vi "GDSProject_GetAllClasses.vi"(1 "AnyProjectItemRefnum":refnum<vi>, 2 "TreeControlRef":refnum<vi>, 3 "ClassProviderName":string, 4 "RootParentTag":string="LabVIEW Object", 5 "error In":errorcluster, 6 "Interfaces(False)":bool, 8 "ClassFilter":string) -> (15 "ClassPaths":path[](array[path]), 16 "ClassTags":string[](array[string]), 19 "error out":errorcluster)   [LabVIEW 2020]
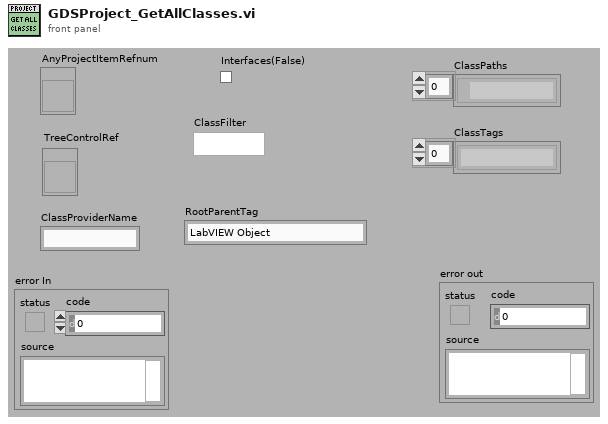
[diagram p1: front panel]
types:
  T1 = cluster{"Classes":refnum<vi>[], "Parents":refnum<vi>[], "ClassIneritance":cluster{string[]}[], "ClassTags":string[], "ClassPaths":path[], "ClassNames":string[]}
  T2 = typedef "GDSLvCLass_ClassSettingsType.ctl" = cluster{"ClassProviderName":string, "ClassTemplateUsed":string, "ClassTemplateVersion":string, "ClassDescription":string, "PlugIns":T3[], "ConnectorPanePattern":string}
  T3 = typedef "GDSLvClass_PlugIn.ctl" = cluster{"Type":T4, "ID":string, "Version":string, "Path":path, "Name":string, "Data":variant}
  T4 = typedef "GDSLvClass_PlugInTypes.ctl" = enum16{"DesignPattern", "MethodTypes"}
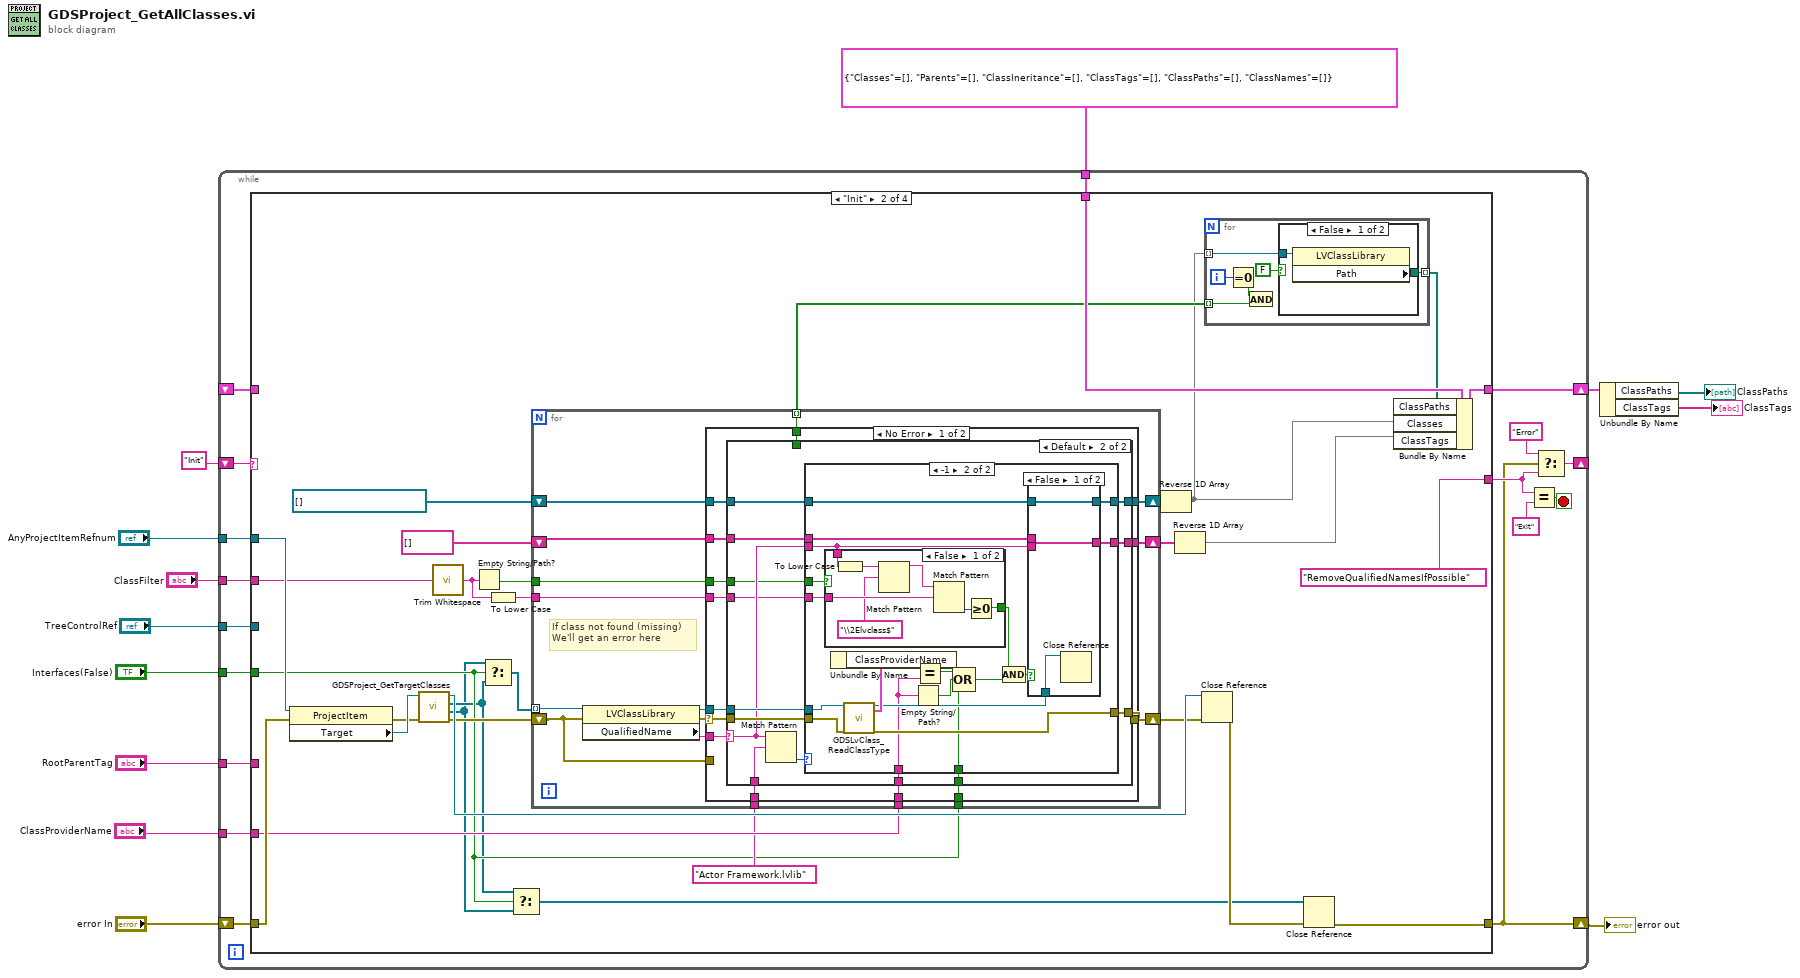
[diagram p0: block diagram]
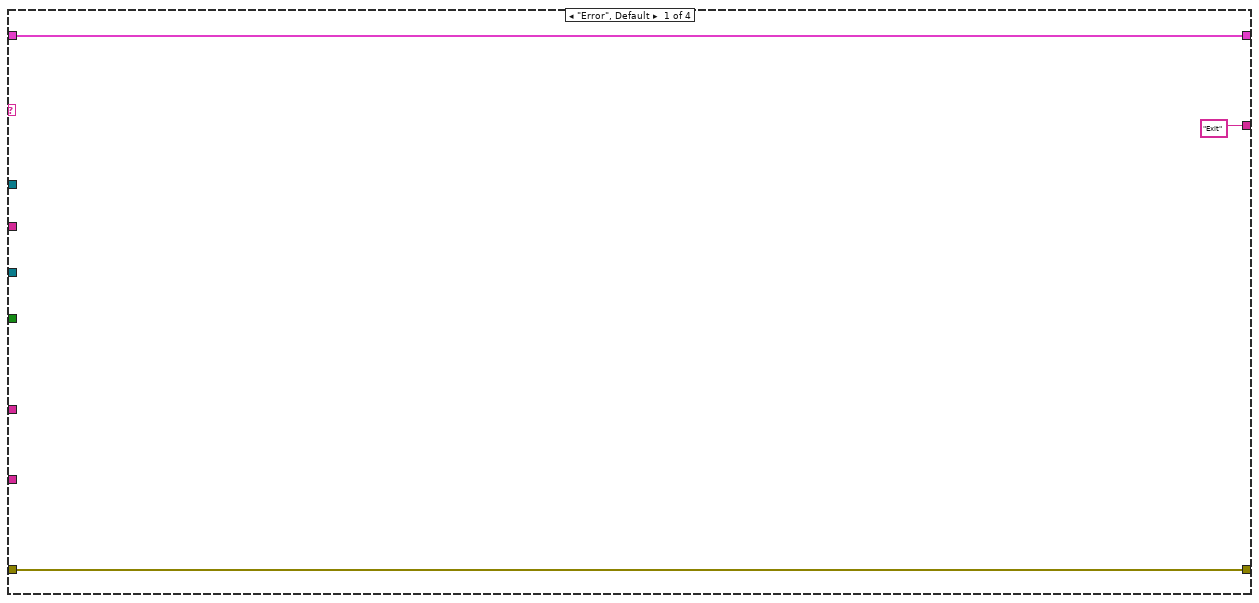
[diagram p2: hidden frame]
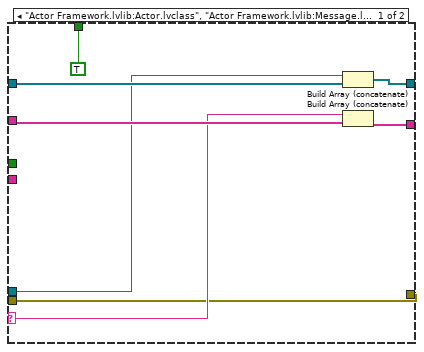
[diagram p4: hidden frame]
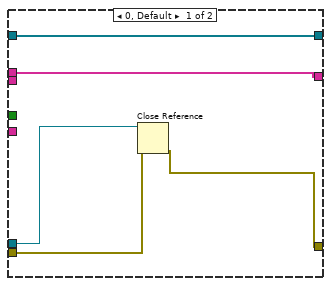
[diagram p5: hidden frame]
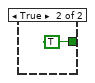
[diagram p6: hidden frame]
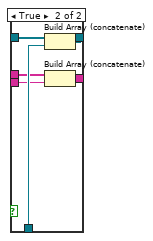
[diagram p7: hidden frame]
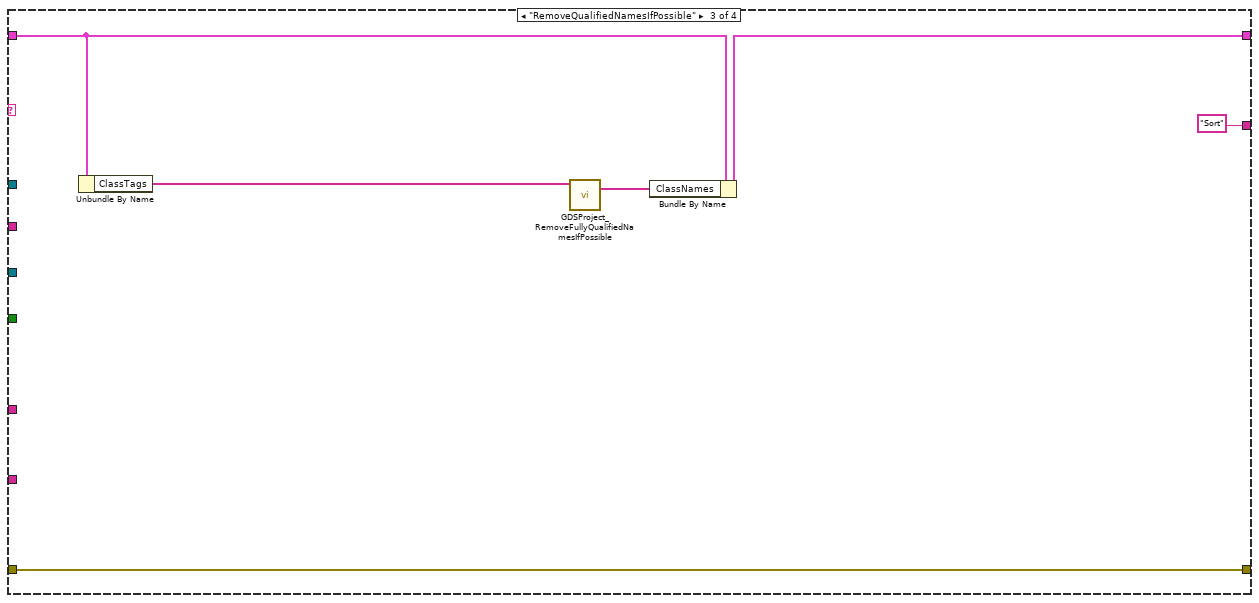
[diagram p9: hidden frame]
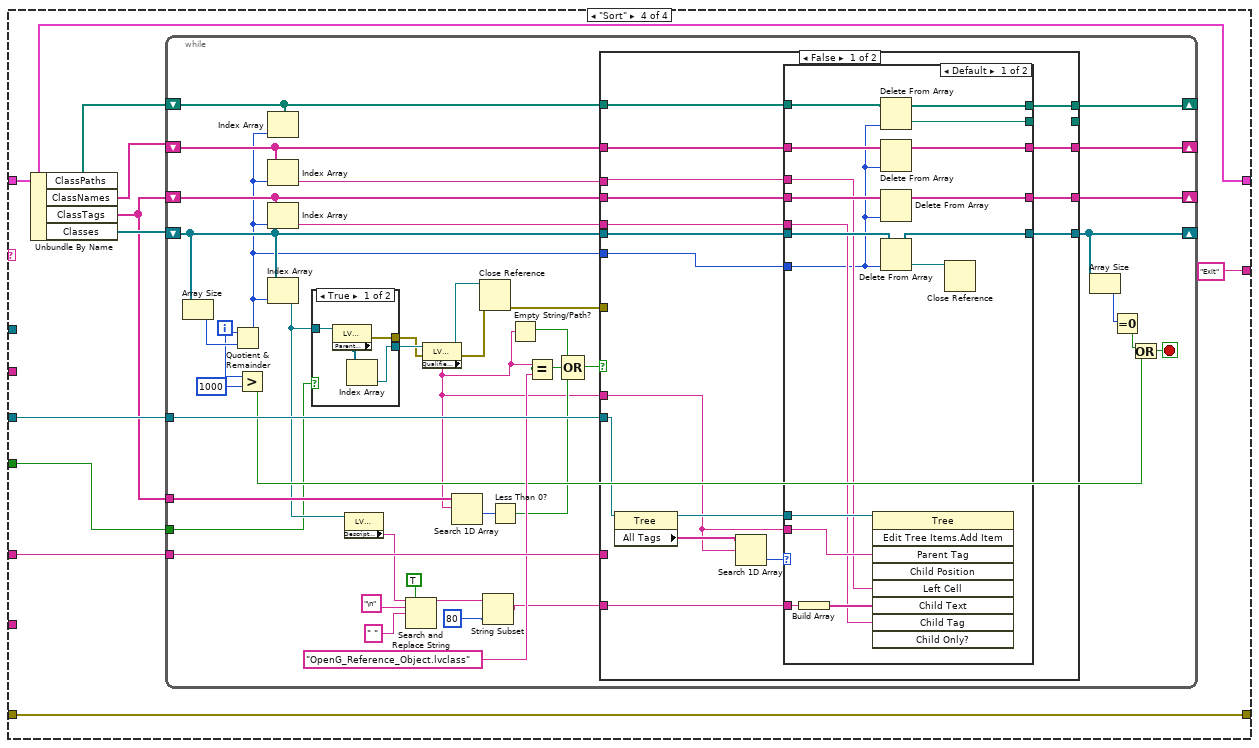
[diagram p10: hidden frame]
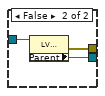
[diagram p11: hidden frame]
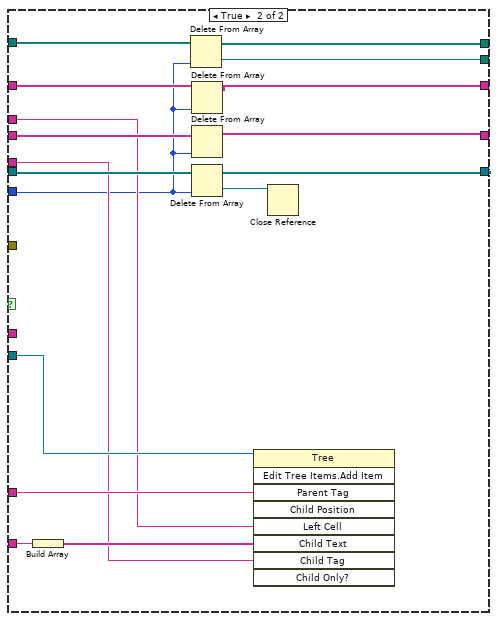
[diagram p13: hidden frame]
diagram:
  n1 = while {
    shift-right: [w23] -> w2
    shift-left: "error In" -> [w30]
    shift-right: [w28] -> _
    shift-left: "Init" -> [w29]
    shift-right: [w22] -> w6
    shift-left: _ -> [w21]
    tunnel: "AnyProjectItemRefnum" -> [w20]
    tunnel: T1 {"Classes"=[], "Parents"=[], "ClassIneritance"=[], "ClassTags"=[], "ClassPaths"=[], "ClassNames"=[]} -> [w19]
    tunnel: "ClassProviderName" -> [w18]
    tunnel: "TreeControlRef" -> [w17]
    tunnel: "RootParentTag" -> [w16]
    tunnel: "Interfaces(False)" -> [w15]
    tunnel: "ClassFilter" -> [w14]
    stop <- w27 stop-if-true
    n2 = case shown="\"Init\"" w29 {
      tunnel: w30 -> [w33 w60 w170 w182]
      tunnel: [w33 w39 w170 w182] -> w23
      tunnel: ["Exit" "RemoveQualifiedNamesIfPossible" "Sort" "Exit"] -> w24
      tunnel: [w31 w58 w172 w180] -> w22
      tunnel: w21 -> [w31 _ w174 w180]
      tunnel: w20 -> [_ w62 _ _]
      tunnel: w19 -> [_ w59 _ _]
      tunnel: w18 -> [_ w57 _ _]
      tunnel: w17 -> [_ _ _ w181]
      tunnel: w16 -> [_ _ _ w183]
      tunnel: w15 -> [_ w43 _ w176]
      tunnel: w14 -> [_ w37 _ _]
      frame "Error", Default {
      }
      frame "Init" {
        n3 = property class="ProjectItem"(reference=w62, error in=w60) -> (error out=w50:errorcluster, "Target"=w51:refnum<vi>)  [unwired: 1 out]
        n4 = call "GDSProject_GetTargetClasses.vi"("error in (no error)"=w50, "TargetItem in"=w51) -> ("error out"=w61:errorcluster, "LvInterfaces"=w41:refnum<vi>[], "LvClasses"=w42:refnum<vi>[], "TargetItem out"=w63:refnum<vi>)  [unwired: 4 in, 2 out]
        n5 = call <vilib>:"Trim Whitespace.vi"("string"=w37) -> ("trimmed string"=w35:string)  [unwired: 1 in]
        n6 = Empty String/Path?(string/path=w35) -> (empty?=w36:bool)
        n7 = Select(t=w41, s=w43, f=w42) -> (s? t:f=w44:refnum<vi>[])
        n8 = To Lower Case(string=w35) -> (all lower case string=w34:string)
        n9 = Select(t=w42, s=w43, f=w41) -> (s? t:f=w38:refnum<vi>[])
        n10 = for {
          tunnel: w44 -> [w77] mode=indexing
          shift-right: [w78] -> w53
          shift-left: refnum<vi>[] [] -> [w88]
          shift-right: [w87] -> w49
          shift-left: w61 -> [w75]
          tunnel: w57 -> [w86]
          shift-right: [w85] -> w54
          shift-left: string[] [] -> [w84]
          tunnel: [w80] -> w48 mode=indexing
          tunnel: "Actor Framework.lvlib" ("Type") -> [w79]
          tunnel: w43 -> [w76]
          tunnel: w36 -> [w74]
          tunnel: w34 -> [w73]
          # "If class not found (missing)\nWe'll get an error here"
          n11 = property class="LVClassLibrary"(reference=w77, error in=w75) -> (reference out=w83:refnum<vi>, error out=w82:errorcluster, "QualifiedName"=w81:string)
          n12 = case shown="No Error" w82 {
            selector: w82 -> [w96 _]
            tunnel: w88 -> [w102 w167]
            tunnel: [w101 w169] -> w87
            tunnel: w86 -> [w100 _]
            tunnel: [w99 w168] -> w85
            tunnel: w84 -> [w98 w168]
            tunnel: w83 -> [w97 _]
            tunnel: w81 -> [w95 _]
            tunnel: [w94 _] -> w80
            tunnel: w79 -> [w93 _]
            tunnel: [w92 w167] -> w78
            tunnel: w76 -> [w91 _]
            tunnel: w75 -> [_ w169]
            tunnel: w74 -> [w90 _]
            tunnel: w73 -> [w89 _]
            frame No Error {
              n13 = case shown="Default" w95 {
                selector: w95 -> [w106 w114]
                tunnel: [w110 w115] -> w92
                tunnel: w102 -> [w104 w124]
                tunnel: [w105 w123] -> w101
                tunnel: w100 -> [_ w122]
                tunnel: [w109 w121] -> w99
                tunnel: w98 -> [w108 w120]
                tunnel: w97 -> [w103 w119]
                tunnel: w96 -> [w105 w118]
                tunnel: [TRUE _] -> w94
                tunnel: w93 -> [_ w117]
                tunnel: w91 -> [_ w113]
                tunnel: w90 -> [_ w112]
                tunnel: w89 -> [_ w111]
                frame "Actor Framework.lvlib:Actor.lvclass", "Actor Framework.lvlib:Message.lvclass" {
                  n14 = Build Array (concatenate)(w103, w104) -> (w110:refnum<vi>[])
                  n15 = Build Array (concatenate)(w106, w108) -> (w109:string[])
                }
                frame Default {
                  n16 = Match Pattern(string=w114, regular expression=w117) -> (offset past match=w116:i32)  [unwired: 1 in, 3 out]
                  n17 = case shown="-1" w116 {
                    tunnel: [w129 w149] -> w115
                    tunnel: w124 -> [w129 w148]
                    tunnel: [w125 w145] -> w123
                    tunnel: w122 -> [_ w143]
                    tunnel: [w128 w140] -> w121
                    tunnel: w120 -> [w128 w139]
                    tunnel: w119 -> [w127 w138]
                    tunnel: w118 -> [w126 w137]
                    tunnel: w114 -> [_ w131]
                    tunnel: w113 -> [_ w136]
                    tunnel: w112 -> [_ w133]
                    tunnel: w111 -> [_ w130]
                    frame 0, Default {
                      n18 = Close Reference(reference=w127, error in (no error)=w126) -> (error out=w125:errorcluster)
                    }
                    frame -1 {
                      n19 = case shown="False" w133 {
                        tunnel: [w153 TRUE] -> w132
                        tunnel: w131 -> [w156 _]
                        tunnel: w130 -> [w155 _]
                        frame False {
                          n20 = To Lower Case(string=w156) -> (all lower case string=w151:string)
                          n21 = Match Pattern(string=w151, regular expression="\\2Elvclass$") -> (before substring=w150:string)  [unwired: 1 in, 3 out]
                          n22 = Match Pattern(string=w150, regular expression=w155) -> (offset past match=w154:i32)  [unwired: 1 in, 3 out]
                          n23 = Greater Or Equal To 0?(x=w154) -> (x >= 0?=w153:bool)
                        }
                        frame True {
                        }
                      }
                      n24 = call "GDSLvClass_ReadClassType.vi"("Class Refnum In"=w138, "error in (no error)"=w137) -> ("Class Refnum Out"=w146:refnum<vi>, "ClassSettings"=w147:T2, "error out"=w145:errorcluster)  [unwired: 15 in]
                      n25 = Unbundle By Name(w147) -> ("ClassProviderName"=w144:string)
                      n26 = Empty String/Path?(string/path=w143) -> (empty?=w141:bool)
                      n27 = Equal?(x=w144, y=w143) -> (x = y?=w142:bool)
                      n28 = Compound Arithmetic op=OR(w142, w141, w136) -> (w135:bool)
                      n29 = Compound Arithmetic op=AND(w132, w135) -> (w134:bool)
                      n30 = case shown="False" w134 {
                        tunnel: [w160 w166] -> w149
                        tunnel: w148 -> [w160 w165]
                        tunnel: w146 -> [w159 w164]
                        tunnel: [w158 w163] -> w140
                        tunnel: w139 -> [w158 w162]
                        tunnel: w131 -> [_ w161]
                        frame False {
                          n31 = Close Reference(reference=w159) -> ()  [unwired: 1 in, 1 out]
                        }
                        frame True {
                          n32 = Build Array (concatenate)(w165, w164) -> (w166:refnum<vi>[])
                          n33 = Build Array (concatenate)(w162, w161) -> (w163:string[])
                        }
                      }
                    }
                  }
                }
              }
            }
            frame Error {
            }
          }
        }
        n34 = Reverse 1D Array(array=w53) -> (reversed array=w47:refnum<vi>[])
        n35 = Reverse 1D Array(array=w54) -> (reversed array=w46:string[])
        n36 = Close Reference(reference=w63, error in (no error)=w49) -> (error out=w40:errorcluster)
        n37 = for {
          tunnel: w47 -> [w70] mode=indexing
          tunnel: [w69] -> w52 mode=indexing
          tunnel: w48 -> [w66] mode=indexing
          i -> [w68]
          n38 = Equal To 0?(x=w68) -> (x = 0?=w67:bool)
          n39 = And(x=w67, y=w66) -> ()  [unwired: 1 out]
          n40 = case shown="False" FALSE {
            tunnel: w70 -> [w72 _]
            tunnel: [w71 _] -> w69
            frame False {
              n41 = property class="LVClassLibrary"(reference=w72) -> ("Path"=w71:path)  [unwired: 1 in, 2 out]
            }
            frame True {
            }
          }
        }
        n42 = Close Reference(reference=w38, error in (no error)=w40) -> (error out=w39:errorcluster)
        n43 = Bundle By Name(cluster=w59, "ClassPaths"=w52, "Classes"=w47, "ClassTags"=w46) -> (w58:T1)
      }
      frame "RemoveQualifiedNamesIfPossible" {
        n44 = Unbundle By Name(w174) -> ("ClassTags"=w175:string[])
        n45 = call "GDSProject_RemoveFullyQualifiedNamesIfPossible.vi"("ItemnamesIn"=w175) -> ("ItemnamesOut"=w173:string[])  [unwired: 10 in]
        n46 = Bundle By Name(cluster=w174, "ClassNames"=w173) -> (w172:T1)
      }
      frame "Sort" {
        n47 = Unbundle By Name(w180) -> ("ClassPaths"=w177:path[], "ClassNames"=w179:string[], "ClassTags"=w178:string[], "Classes"=w185:refnum<vi>[])
        n48 = while {
          shift-right: [w225] -> _
          shift-left: w185 -> [w226]
          tunnel: w181 -> [w227]
          tunnel: w183 -> [w222]
          tunnel: w178 -> [w212]
          shift-right: [w203] -> _
          shift-left: w178 -> [w202]
          shift-right: [w199] -> _
          shift-left: w179 -> [w200]
          shift-right: [w187] -> _
          shift-left: w177 -> [w188]
          tunnel: w176 -> [w186]
          i -> [w215]
          stop <- w216 stop-if-true
          n49 = Array Size(array=w226) -> (size(s)=w223:i32)
          n50 = Quotient & Remainder(x=w215, y=w223) -> (x-y*floor(x/y)=w189:i32)  [unwired: 1 out]
          n51 = Greater?(x=w215, y=1000) -> (0:w213:bool)
          n52 = Index Array(array=w188, index=w189) -> ()  [unwired: 1 out]
          n53 = Index Array(array=w200, index=w189) -> (element=w197:string)
          n54 = Index Array(array=w202, index=w189) -> (element=w201:string)
          n55 = Index Array(array=w226, index=w189) -> (element=w196:refnum<vi>)
          n56 = case shown="True" w186 {
            tunnel: [w228 w234] -> w204
            tunnel: w196 -> [w231 w233]
            tunnel: [w230 w232] -> w193
            frame True {
              n57 = property class="LVClassLibrary"(reference=w231) -> (error out=w230:errorcluster, "Parent Interfaces"=w229:refnum<vi>[])  [unwired: 1 in, 1 out]
              n58 = Index Array(array=w229) -> (element=w228:refnum<vi>)  [unwired: 1 in]
            }
            frame False {
              n59 = property class="LVClassLibrary"(reference=w233) -> (error out=w232:errorcluster, "Parent"=w234:refnum<vi>)  [unwired: 1 in, 1 out]
            }
          }
          n60 = property class="LVClassLibrary"(reference=w196) -> ("Description"=w198:string)  [unwired: 1 in, 2 out]
          n61 = Search and Replace String(replace all?=TRUE ("replace all? (F)"), input string=w198, search string="\n" ("replace string (\"\")"), replace string=" " ("replace string (\"\")")) -> (result string=w208:string)  [unwired: 4 in, 3 out]
          n62 = property class="LVClassLibrary"(reference=w204, error in=w193) -> (reference out=w195:refnum<vi>, error out=w194:errorcluster, "QualifiedName"=w191:string)
          n63 = Search 1D Array(1D array=w212, element=w191) -> (index of element=w211:i32)  [unwired: 1 in]
          n64 = Close Reference(reference=w195, error in (no error)=w194) -> (error out=w192:errorcluster)
          n65 = String Subset(string=w208, length (rest)=80 ("length (rest)")) -> (substring=w206:string)  [unwired: 1 in]
          n66 = Less Than 0?(x=w211) -> (x < 0?=w210:bool)
          n67 = Empty String/Path?(string/path=w191) -> (empty?=w221:bool)
          n68 = Equal?(x=w191, y="OpenG_Reference_Object.lvclass") -> (x = y?=w219:bool)
          n69 = Compound Arithmetic op=OR(w221, w219, w210) -> (w220:bool)
          n70 = case shown="False" w220 {
            tunnel: w227 -> [w251 w289]
            tunnel: w226 -> [w247 w288]
            tunnel: w189 -> [w246 w275]
            tunnel: [w245 w287] -> w225
            tunnel: w206 -> [w244 w279]
            tunnel: w222 -> [_ w284]
            tunnel: w202 -> [w243 w283]
            tunnel: [w242 w282] -> w203
            tunnel: w201 -> [w241 w278]
            tunnel: w200 -> [w240 w281]
            tunnel: [w239 w280] -> w199
            tunnel: w197 -> [w238 w277]
            tunnel: w191 -> [w237 _]
            tunnel: w192 -> [_ _]
            tunnel: w188 -> [w236 w276]
            tunnel: [w235 w274] -> w187
            tunnel: [_ w273] -> _
            frame False {
              n71 = property class="Tree"(reference=w251) -> (reference out=w248:refnum<vi>, "All Tags"=w250:string[])  [unwired: 1 in, 1 out]
              n72 = Search 1D Array(1D array=w250, element=w237) -> (index of element=w249:i32)  [unwired: 1 in]
              n73 = case shown="Default" w249 {
                tunnel: w248 -> [w268 _]
                tunnel: w237 -> [w267 _]
                tunnel: w247 -> [w266 w272]
                tunnel: w246 -> [w253 _]
                tunnel: [w265 w272] -> w245
                tunnel: w244 -> [w263 _]
                tunnel: w243 -> [w261 w271]
                tunnel: [w260 w271] -> w242
                tunnel: w241 -> [w259 _]
                tunnel: w240 -> [w258 w270]
                tunnel: [w257 w270] -> w239
                tunnel: w238 -> [w256 _]
                tunnel: w236 -> [w255 w269]
                tunnel: [w254 w269] -> w235
                tunnel: [w252 _] -> _
                frame Default {
                  n74 = Build Array(w263) -> (w262:string[])
                  n75 = invoke class="Tree" method="Edit Tree Items.Add Item"(reference=w268, "Parent Tag"=w267, "Left Cell"=w256, "Child Text"=w262, "Child Tag"=w259) -> ()  [unwired: 4 in, 9 out]
                  n76 = Delete From Array(array=w255, index=w253) -> (deleted portion=w252:path, array with subset deleted=w254:path[])  [unwired: 1 in]
                  n77 = Delete From Array(array=w258, index=w253) -> (array with subset deleted=w257:string[])  [unwired: 1 in, 1 out]
                  n78 = Delete From Array(array=w261, index=w253) -> (array with subset deleted=w260:string[])  [unwired: 1 in, 1 out]
                  n79 = Delete From Array(array=w266, index=w253) -> (deleted portion=w264:refnum<vi>, array with subset deleted=w265:refnum<vi>[])  [unwired: 1 in]
                  n80 = Close Reference(reference=w264) -> ()  [unwired: 1 in, 1 out]
                }
                frame -1 {
                }
              }
            }
            frame True {
              n81 = Build Array(w279) -> (w285:string[])
              n82 = Delete From Array(array=w276, index=w275) -> (deleted portion=w273:path, array with subset deleted=w274:path[])  [unwired: 1 in]
              n83 = Delete From Array(array=w281, index=w275) -> (array with subset deleted=w280:string[])  [unwired: 1 in, 1 out]
              n84 = Delete From Array(array=w283, index=w275) -> (array with subset deleted=w282:string[])  [unwired: 1 in, 1 out]
              n85 = Delete From Array(array=w288, index=w275) -> (deleted portion=w286:refnum<vi>, array with subset deleted=w287:refnum<vi>[])  [unwired: 1 in]
              n86 = invoke class="Tree" method="Edit Tree Items.Add Item"(reference=w289, "Parent Tag"=w284, "Left Cell"=w277, "Child Text"=w285, "Child Tag"=w278) -> ()  [unwired: 4 in, 9 out]
              n87 = Close Reference(reference=w286) -> ()  [unwired: 1 in, 1 out]
            }
          }
          n88 = Array Size(array=w225) -> (size(s)=w224:i32)
          n89 = Equal To 0?(x=w224) -> (x = 0?=w217:bool)
          n90 = Or(x=w217, y=w213) -> (x .or. y?=w216:bool)
        }
      }
    }
    n91 = Equal?(x=w24, y="Exit") -> (x = y?=w27:bool)
    n92 = Select(t="Error", s=w23, f=w24) -> (s? t:f=w28:string)
  }
  "error out" <- w2
  n93 = Unbundle By Name(w6) -> ("ClassPaths"=→"ClassPaths":path[], "ClassTags"=→"ClassTags":string[])
